vi "Determine Path Points.vi"(8 "error in (no error)":errorcluster, 11 "Tool Path in":refnum<class "Tool Path.lvclass">) -> (0 "error out":errorcluster, 2 "Points":T1[](array[typedef]), 3 "Tool Path out":refnum<class "Tool Path.lvclass">)   [LabVIEW 2019, in "Tool Path.lvclass"]
uses:
  Tool Path.lvclass
  Parse/PathCommands/Point.ctl
  Parse/ParsePaths/Path.lvclass/Path.ctl
  Settings/Path Settings/Path Settings.lvclass/Path Settings.ctl
  Parse/PathCommands/PathCommands.lvclass
  Parse/ParsePaths/Path.lvclass
  Settings/Path Settings/Path Settings.lvclass
panel:
  in  "Numeric":i32=40
  out "XY Graph 2":cluster{"X":dbl, "Y":dbl}[](graph)
  out "Points Arrays":cluster{"X":dbl[], "Y":dbl[]}
  out "x-y":u32
  out "XY Graph":cluster{"X":dbl, "Y":dbl}[](graph)
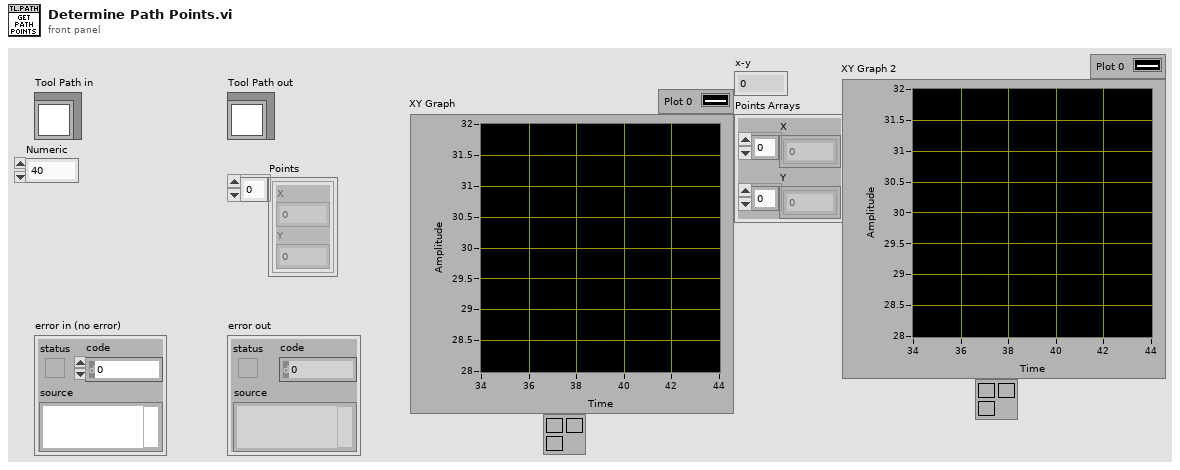
[diagram p1: front panel]
types:
  T1 = typedef "PathCommands.lvclass/Point.ctl" = cluster{"X":dbl, "Y":dbl}
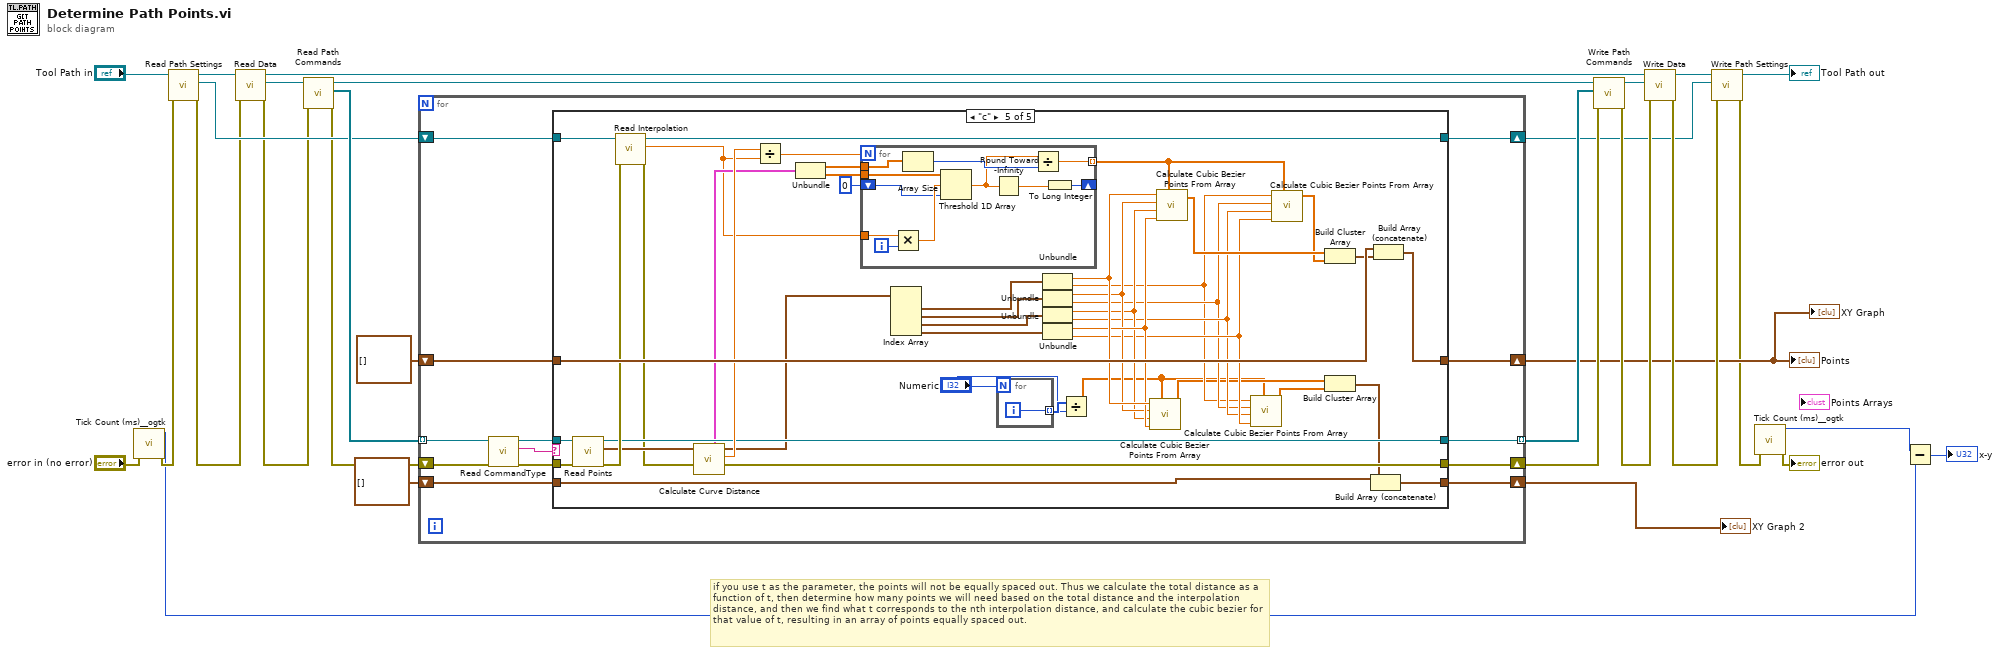
[diagram p0: block diagram]
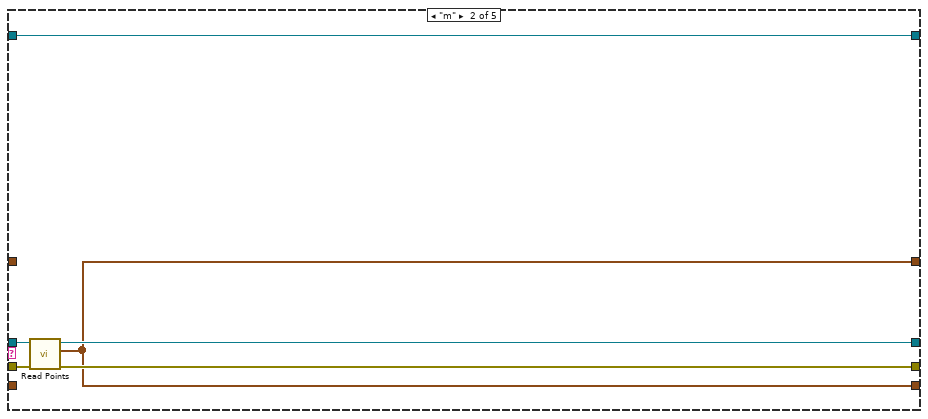
[diagram p3: hidden frame]
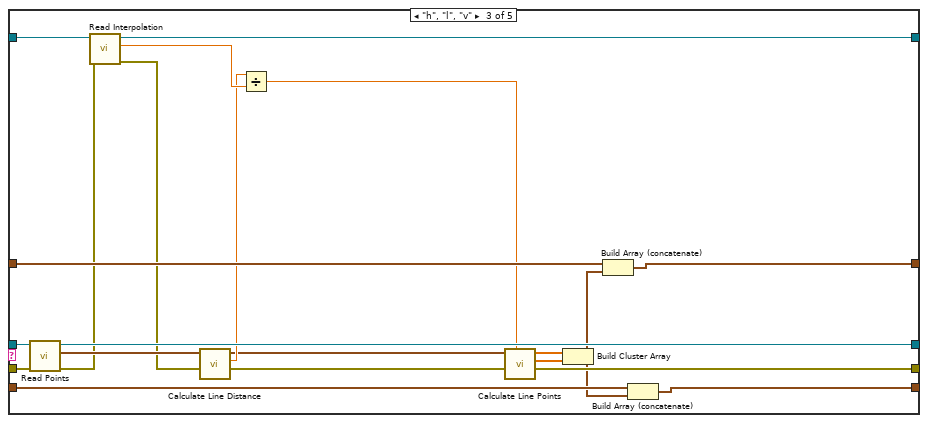
[diagram p4: hidden frame]
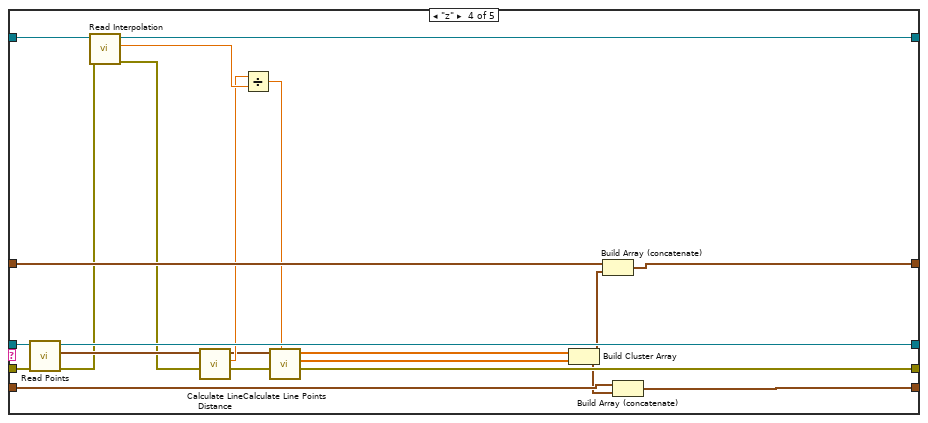
[diagram p5: hidden frame]
diagram:
  # "if you use t as the parameter, the points will not be equally spaced out. Thus we calculate the total distance as a function of t, then determine how many points we will need based on the total distance and the interpolation distance, and then we find what t corresponds to the nth interpolation distance, and calculate the cubic bezier for that value of t, resulting in an array of points equally spaced out."
  n1 = call <userlib>:"Tick Count (ms)__ogtk.vi"("error in (no error)"="error in (no error)") -> ("error out"=w8:errorcluster, "millisecond timer value"=w4:u32)  [unwired: 9 in]
  n2 = call-dynamic "Read Path Settings.vi"("error in (no error)"=w8, "Tool Path in"="Tool Path in") -> ("error out"=w19:errorcluster, "Path Settings.lvclass"=w20:refnum<class "Path Settings.lvclass">, "Tool Path out"=w24:refnum<class "Tool Path.lvclass">)  [unwired: 7 in]
  n3 = call-dynamic "Read Data.vi"("error in (no error)"=w19, "Tool Path in"=w24) -> ("error out"=w18:errorcluster, "Path.lvclass"=w23:refnum<class "Path.lvclass">, "Tool Path out"=w21:refnum<class "Tool Path.lvclass">)  [unwired: 7 in]
  n4 = call "Read Path Commands.vi"("error in (no error)"=w18, "Path in"=w23) -> ("error out"=w17:errorcluster, "Path Commands"=w28:refnum<class "PathCommands.lvclass">[], "Path out"=w29:refnum<class "Path.lvclass">)  [unwired: 7 in]
  n5 = for {
    shift-right: [w33] -> w15
    shift-left: w17 -> [w32]
    tunnel: w28 -> [w40] mode=indexing
    tunnel: [w42] -> w27 mode=indexing
    shift-right: [w35] -> w10
    shift-left: T1[] [] ("Points") -> [w38]
    shift-right: [w36] -> w12
    shift-left: w20 -> [w37]
    shift-right: [w31] -> w2
    shift-left: cluster{dbl, dbl}[] [] -> [w30]
    n6 = call-dynamic "Read CommandType.vi"("error in (no error)"=w32, "PathCommands in"=w40) -> ("error out"=w39:errorcluster, "CommandType"=w34:string, "PathCommands out"=w41:refnum<class "PathCommands.lvclass">)  [unwired: 7 in]
    n7 = case shown="\"c\"" w34 {
      tunnel: [w47 w51 w59 w82 w121] -> w33
      tunnel: w39 -> [w47 w50 w72 w93 w137]
      tunnel: [w46 w52 w73 w94 w130] -> w42
      tunnel: w41 -> [w46 w53 w74 w95 w138]
      tunnel: [w45 w48 w68 w89 w133] -> w35
      tunnel: w38 -> [w45 _ w67 w88 w134]
      tunnel: w37 -> [w44 w49 w70 w91 w135]
      tunnel: [w44 w49 w71 w92 w136] -> w36
      tunnel: [w43 w48 w56 w77 w100] -> w31
      tunnel: w30 -> [w43 _ w55 w76 w99]
      frame Default {
      }
      frame "m" {
        n8 = call-dynamic "Read Points.vi"("error in (no error)"=w50, "PathCommands in"=w53) -> ("error out"=w51:errorcluster, "Points"=w48:T1[], "PathCommands out"=w52:refnum<class "PathCommands.lvclass">)  [unwired: 7 in]
      }
      frame "h", "l", "v" {
        # "Create interpolation VI\nCreate Distance VI"
        n9 = call-dynamic "Read Points.vi"("error in (no error)"=w72, "PathCommands in"=w74) -> ("error out"=w62:errorcluster, "Points"=w66:T1[], "PathCommands out"=w73:refnum<class "PathCommands.lvclass">)  [unwired: 7 in]
        n10 = call "Read Interpolation.vi"("error in (no error)"=w62, "Path Settings in"=w70) -> ("error out"=w61:errorcluster, "Interpolation"=w69:dbl, "Path Settings out"=w71:refnum<class "Path Settings.lvclass">)  [unwired: 7 in]
        n11 = call "Calculate Line Distance.vi"("error in (no error)"=w61, "Points"=w66) -> ("error out"=w60:errorcluster, "Distance"=w65:dbl, "Points Out"=w64:T1[])  [unwired: 7 in]
        n12 = Divide(x=w65, y=w69) -> (x/y=w63:dbl)
        n13 = call "Calculate Line Points.vi"("Iterations"=w63, "error in (no error)"=w60, "Points"=w64) -> ("error out"=w59:errorcluster, "Y"=w58:dbl[], "X"=w57:dbl[])  [unwired: 6 in]
        n14 = Build Cluster Array(w57, w58) -> (w54:cluster{"X":dbl, "Y":dbl}[])
        n15 = Build Array (concatenate)(w67, w54) -> (w68:T1[])
        n16 = Build Array (concatenate)(w55, w54) -> (w56:T1[])
      }
      frame "z" {
        # "Create interpolation VI\nCreate Distance VI"
        n17 = call-dynamic "Read Points.vi"("error in (no error)"=w93, "PathCommands in"=w95) -> ("error out"=w80:errorcluster, "Points"=w87:T1[], "PathCommands out"=w94:refnum<class "PathCommands.lvclass">)  [unwired: 7 in]
        n18 = call "Read Interpolation.vi"("error in (no error)"=w80, "Path Settings in"=w91) -> ("error out"=w81:errorcluster, "Interpolation"=w90:dbl, "Path Settings out"=w92:refnum<class "Path Settings.lvclass">)  [unwired: 7 in]
        n19 = call "Calculate Line Distance.vi"("error in (no error)"=w81, "Points"=w87) -> ("error out"=w83:errorcluster, "Distance"=w86:dbl, "Points Out"=w84:T1[])  [unwired: 7 in]
        n20 = Divide(x=w86, y=w90) -> (x/y=w85:dbl)
        n21 = call "Calculate Line Points.vi"("Iterations"=w85, "error in (no error)"=w83, "Points"=w84) -> ("error out"=w82:errorcluster, "Y"=w78:dbl[], "X"=w79:dbl[])  [unwired: 6 in]
        n22 = Build Cluster Array(w79, w78) -> (w75:cluster{"X":dbl, "Y":dbl}[])
        n23 = Build Array (concatenate)(w88, w75) -> (w89:T1[])
        n24 = Build Array (concatenate)(w76, w75) -> (w77:T1[])
      }
      frame "c" {
        n25 = call-dynamic "Read Points.vi"("error in (no error)"=w137, "PathCommands in"=w138) -> ("error out"=w131:errorcluster, "Points"=w129:T1[], "PathCommands out"=w130:refnum<class "PathCommands.lvclass">)  [unwired: 7 in]
        n26 = call "Read Interpolation.vi"("error in (no error)"=w131, "Path Settings in"=w135) -> ("error out"=w122:errorcluster, "Interpolation"=w125:dbl, "Path Settings out"=w136:refnum<class "Path Settings.lvclass">)  [unwired: 7 in]
        n27 = call "Calculate Curve Distance.vi"("error in (no error)"=w122, "Points"=w129) -> ("error out"=w121:errorcluster, "Length"=w132:dbl, "Points Out"=w117:T1[], "Distance vs t"=w127:cluster{"t":dbl[], "Distance":dbl[]})  [unwired: 6 in]
        n28 = Divide(x=w132, y=w125) -> (x/y=w128:dbl)
        n29 = Unbundle(w127) -> ("t"=w124:dbl[], "Distance"=w126:dbl[])
        n30 = for {
          N: w128 -> [_]
          tunnel: w126 -> [w148]
          tunnel: w125 -> [w149]
          tunnel: w124 -> [w144]
          shift-right: [w146] -> _
          shift-left: 0 -> [w145]
          tunnel: [w142] -> w115 mode=indexing
          i -> [w150]
          n31 = Multiply(x=w149, y=w150) -> (x*y=w147:dbl)
          n32 = Array Size(array=w144) -> (size(s)=w143:i32)
          n33 = Threshold 1D Array(1:w145, 2:w147, 3:w148) -> (0:w141:dbl)
          n34 = Round Toward -Infinity(1:w141) -> (0:w140:dbl)
          n35 = Divide(x=w141, y=w143) -> (x/y=w142:dbl)
          n36 = To Long Integer(number=w140) -> (32bit integer=w146:i32)
        }
        n37 = Index Array(array=w117) -> (element #1=w116:T1, element #2=w118:T1, element #3=w119:T1, element #4=w120:T1)  [unwired: 4 in]
        n38 = for {
          N: "Numeric" -> [_]
          tunnel: [w139] -> w98 mode=indexing
          i -> [w139]
        }
        n39 = Unbundle(w116) -> ("X"=w111:dbl, "Y"=w104:dbl)
        n40 = Unbundle(w118) -> ("X"=w109:dbl, "Y"=w105:dbl)
        n41 = Unbundle(w119) -> ("X"=w108:dbl, "Y"=w106:dbl)
        n42 = Unbundle(w120) -> ("X"=w110:dbl, "Y"=w107:dbl)
        n43 = Divide(x=w98, y="Numeric") -> (x/y=w97:dbl[])
        n44 = call "Calculate Cubic Bezier Points From Array.vi"("t"=w97, "d"=w110, "c"=w108, "b"=w109, "a"=w111) -> ("f(t)"=w103:dbl[])  [unwired: 6 in]
        n45 = call "Calculate Cubic Bezier Points From Array.vi"("t"=w115, "d"=w110, "c"=w108, "b"=w109, "a"=w111) -> ("f(t)"=w113:dbl[])  [unwired: 6 in]
        n46 = call "Calculate Cubic Bezier Points From Array.vi"("t"=w97, "d"=w107, "c"=w106, "b"=w105, "a"=w104) -> ("f(t)"=w102:dbl[])  [unwired: 6 in]
        n47 = call "Calculate Cubic Bezier Points From Array.vi"("t"=w115, "d"=w107, "c"=w106, "b"=w105, "a"=w104) -> ("f(t)"=w112:dbl[])  [unwired: 6 in]
        n48 = Build Cluster Array(w113, w112) -> (w114:cluster{dbl, dbl}[])
        n49 = Build Cluster Array(w103, w102) -> (w101:cluster{dbl, dbl}[])
        n50 = Build Array (concatenate)(w99, w101) -> (w100:T1[])
        n51 = Build Array (concatenate)(w134, w114) -> (w133:T1[])
      }
    }
  }
  "Points" <- w10
  "XY Graph" <- w10
  "XY Graph 2" <- w2
  n52 = call "Write Path Commands.vi"("error in (no error)"=w15, "Path Commands"=w27, "Path in"=w29) -> ("error out"=w13:errorcluster, "Path out"=w22:refnum<class "Path.lvclass">)  [unwired: 7 in]
  n53 = call-dynamic "Write Data.vi"("error in (no error)"=w13, "Path.lvclass"=w22, "Tool Path in"=w21) -> ("error out"=w14:errorcluster, "Tool Path out"=w16:refnum<class "Tool Path.lvclass">)  [unwired: 7 in]
  n54 = call-dynamic "Write Path Settings.vi"("error in (no error)"=w14, "Path Settings.lvclass"=w12, "Tool Path in"=w16) -> ("error out"=w7:errorcluster, "Tool Path out"=→"Tool Path out":refnum<class "Tool Path.lvclass">)  [unwired: 7 in]
  n55 = call <userlib>:"Tick Count (ms)__ogtk.vi"("error in (no error)"=w7) -> ("error out"=→"error out":errorcluster, "millisecond timer value"=w5:u32)  [unwired: 9 in]
  n56 = Subtract(x=w5, y=w4) -> (x-y=→"x-y":u32)
